vi "ReadAOs.vi"(7 "GroveConnector":enum16{"A0", "A1", "A2"}(ring), 8 "error in (no error)":errorcluster, 11 "Session in":refnum<class "Session.lvclass">) -> (0 "error out":errorcluster, 1 "Duty Cycle %":sgl=0.091836736, 2 "Frequency Hz":sgl=0.001, 3 "Session out":refnum<class "Session.lvclass">)   [LabVIEW 2020]
uses:
  CTI/Session/Session.lvclass
  CTI/GPIO Number.ctl
  CTI/CTI.lvlib
panel:
  # "Input"
  # "Output"
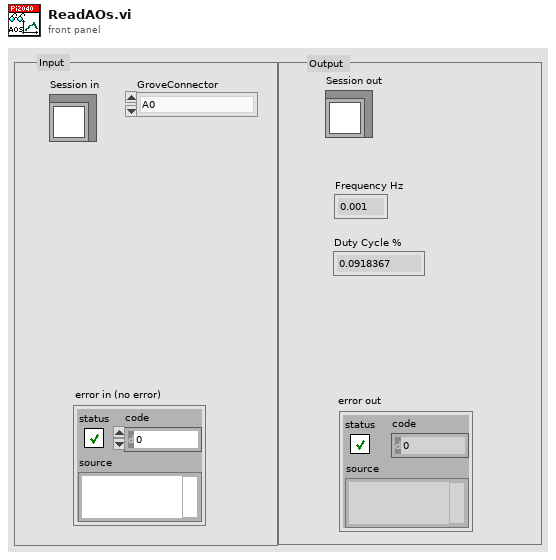
[diagram p1: front panel]
types:
  T1 = typedef "CTI.lvlib/GPIO Number.ctl" = i8
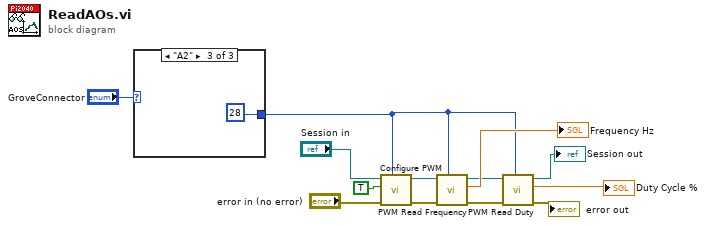
[diagram p0: block diagram]
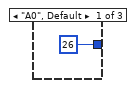
[diagram p2: hidden frame]
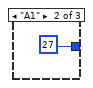
[diagram p3: hidden frame]
diagram:
  n1 = case shown="\"A2\"" "GroveConnector" {
    tunnel: [T1 26 ("GPIO #") T1 27 ("GPIO #") T1 28 ("GPIO #")] -> w5
    frame "A0", Default {
    }
    frame "A1" {
    }
    frame "A2" {
    }
  }
  n2 = call "Configure PWM.vi"("GPIO #"=w5, "error in (no error)"="error in (no error)", "Enable (F)"=TRUE, "Session in"="Session in") -> ("error out"=w8:errorcluster, "Session out"=w9:refnum<class "Session.lvclass">)  [unwired: 6 in]
  n3 = call "PWM Read Frequency.vi"("GPIO #"=w5, "error in (no error)"=w8, "Session in"=w9) -> ("error out"=w3:errorcluster, "Frequency Hz"=→"Frequency Hz":sgl, "Session out"=w6:refnum<class "Session.lvclass">)  [unwired: 6 in]
  n4 = call "PWM Read Duty.vi"("GPIO #"=w5, "error in (no error)"=w3, "Session in"=w6) -> ("error out"=→"error out":errorcluster, "Duty % (0-1)"=→"Duty Cycle %":sgl, "Session out"=→"Session out":refnum<class "Session.lvclass">)  [unwired: 6 in]
